vi "Sample.vi"(8 "错误输入（无错误）":errorcluster, 10 "Time and Data In":T3, 11 "Sample Settings":T1={"设备信息"={"初始索引子集"=[], "模拟信号采集通道"="Dev1", "数字-供电"="", "数字-光控"="", "光控设备"="", "光电设备分离？"=FALSE, "光谱保存路径"=path "", "环数"=0}, "测量控制"={"测头拿起"=FALSE, "起始保存"=FALSE, "测头供电"=TRUE, "测头出光"=TRUE}, "测量"={"每波长测量次数"=5, "波长"=[0, 0, 0, 0, 0, 0], "起始周期"=0, "起始测量周期"=0}, "等待"={"等待时间(s)"=0.0, "等待方式"=FALSE, "每x周期/点等待"=8, "等待时"=enum."无电无光"}, "校准"={"暗电流校准值初值"=[], "温度校准值"=[0.0, 0.0, 0.0, 0.0, 0.0, 0.0, 0.00013, 0.00013, 0.00013, 0.00013, 0.00013, 0.00013], "校准模式"=enum."逐周期"}, "图表相关"={"文件-时间"=""}, "CSM"={"CSM Name"=""}}) -> (0 "error out":errorcluster, 2 "Time and Data Out":T3)   [LabVIEW 2026, in "UI-无创.lvlib" / "Acquisition.lvlib"]
uses:
  Acquisition.lvlib
  Supports/Time and Data_OP.ctl
  Supports/Sample Settings.ctl
  <vilib>/DAQmx/read.llb/DAQmx Read (Analog 2D DBL NChan NSamp).vi
  <vilib>/Analysis/baseanly.llb/Mean (DBL).vi
  <vilib>/DAQmx/create/channels.llb/DAQmx Create Channel (AI-Voltage-Basic).vi
  <vilib>/DAQmx/configure/timing.llb/DAQmx Timing (Sample Clock).vi
  <vilib>/DAQmx/miscellaneous.llb/DAQmx Fill In Error Info.vi
  <vilib>/Analysis/NI_AALBase.lvlib
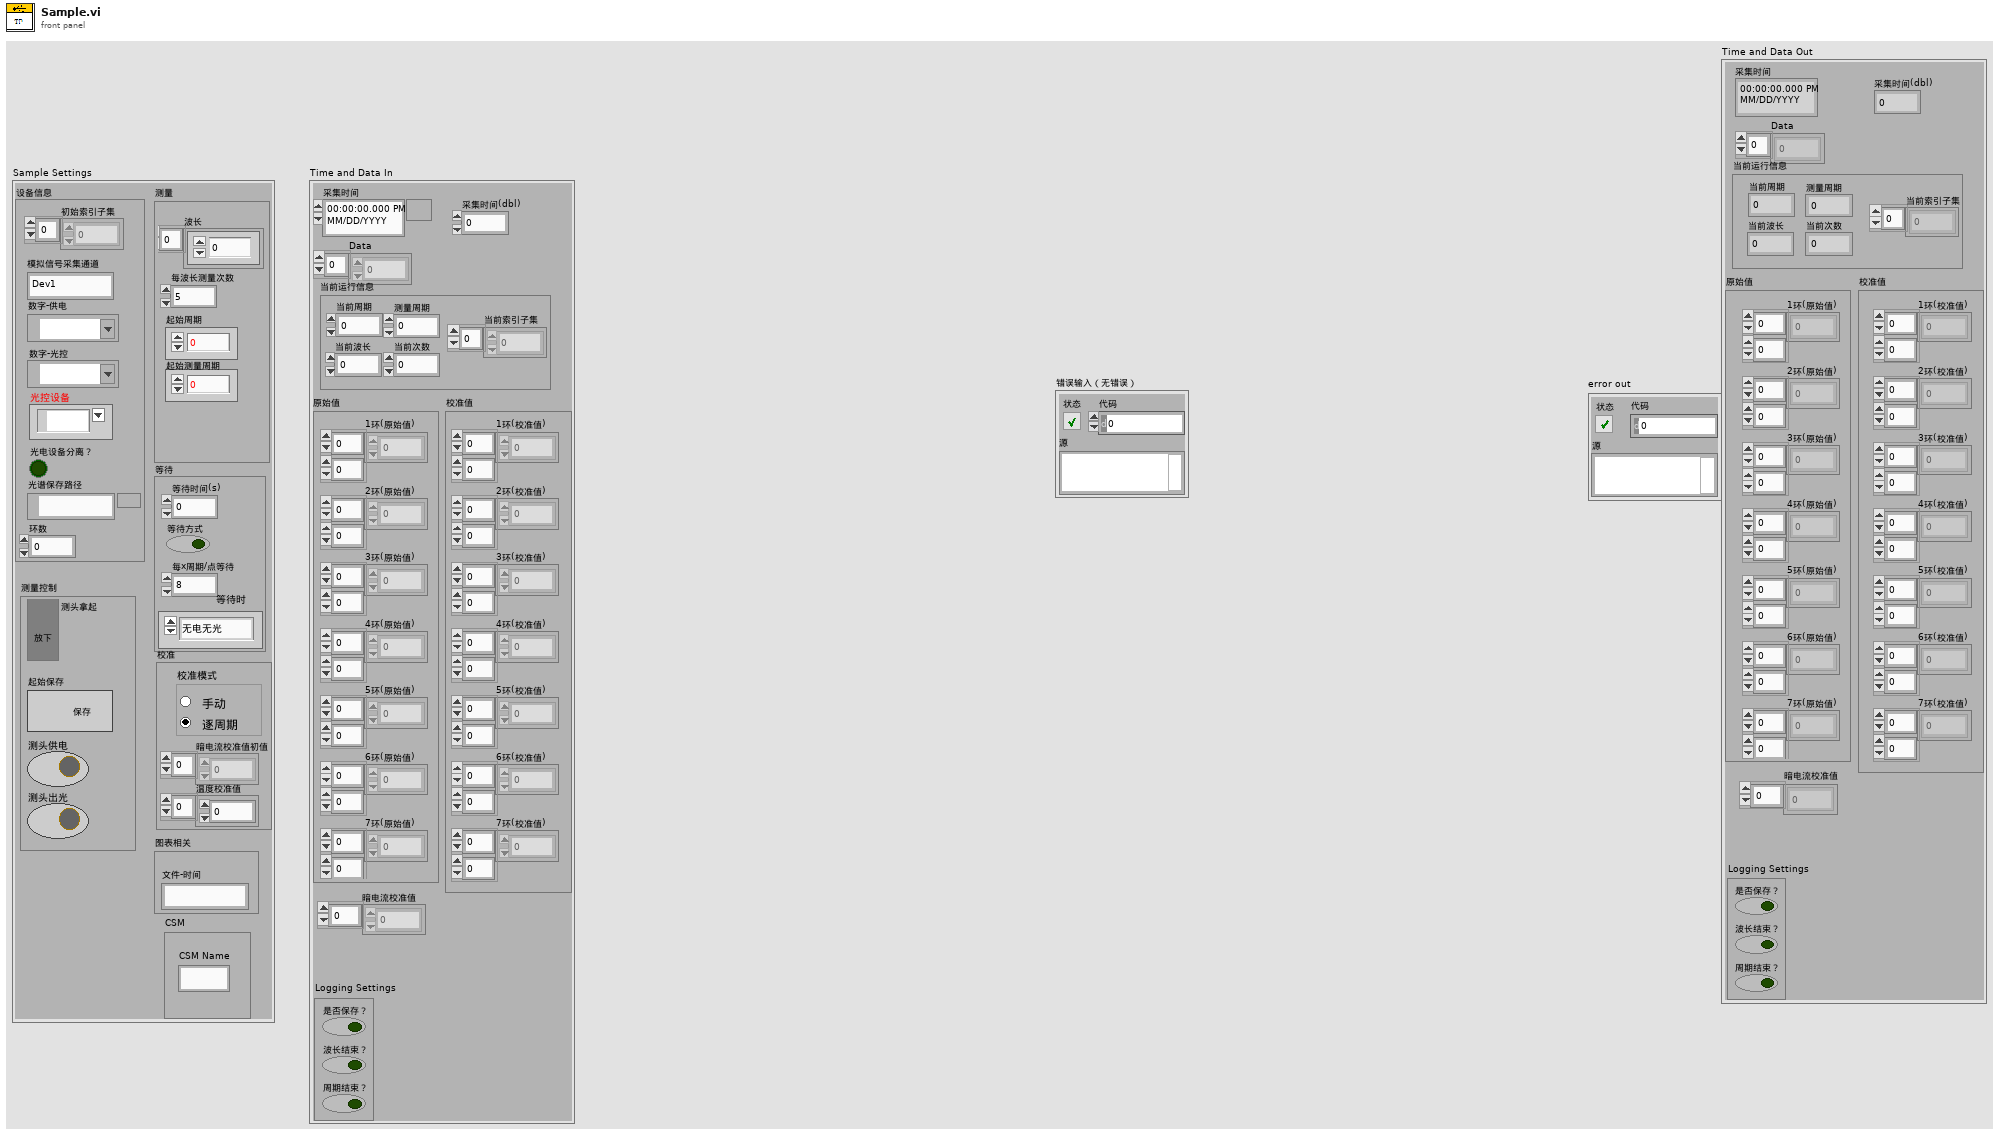
[diagram p1: front panel]
types:
  T1 = typedef "UI-无创.lvlib/Sample Settings.ctl" = cluster{"设备信息":cluster{"初始索引子集":i8[], "模拟信号采集通道":string, "数字-供电":refnum<k21>, "数字-光控":refnum<k21>, "光控设备":tag, "光电设备分离？":bool, "光谱保存路径":path, "环数":u8}, "测量控制":cluster{"测头拿起":bool, "起始保存":bool, "测头供电":bool, "测头出光":bool}, "测量":cluster{"每波长测量次数":i32, "波长":i32[], "起始周期":i32, "起始测量周期":i32}, "等待":cluster{"等待时间(s)":dbl, "等待方式":bool, "每x周期/点等待":i32, "等待时":enum16{"无电无光", "有电无光", "无电有光", "有电有光"}}, "校准":cluster{"暗电流校准值初值":dbl[], "温度校准值":dbl[], "校准模式":T2}, "图表相关":cluster{"文件-时间":string}, "CSM":cluster{"CSM Name":string}}
  T2 = typedef "UI-无创.lvlib/暗电流校准模式.ctl" = enum32{"手动", "逐周期"}
  T3 = typedef "UI-无创.lvlib/Time and Data_OP.ctl" = cluster{"采集时间":timestamp, "采集时间(dbl)":dbl, "Data":dbl[], "当前运行信息":cluster{"当前周期":i32, "当前次数":i32, "测量周期":i32, "当前索引子集":i8[], "当前波长":i32}, "暗电流校准值":dbl[], "Logging Settings":cluster{"是否保存？":bool, "波长结束？":bool, "周期结束？":bool}, "原始值":cluster{"1环(原始值)":dbl[][], "2环(原始值)":dbl[][], "3环(原始值)":dbl[][], "4环(原始值)":dbl[][], "5环(原始值)":dbl[][], "6环(原始值)":dbl[][], "7环(原始值)":dbl[][]}, "校准值":cluster{"1环(校准值)":dbl[][], "2环(校准值)":dbl[][], "3环(校准值)":dbl[][], "4环(校准值)":dbl[][], "5环(校准值)":dbl[][], "6环(校准值)":dbl[][], "7环(校准值)":dbl[][]}}
  T4 = cluster{"Time and Data In":T3, "Sample Settings":T1}
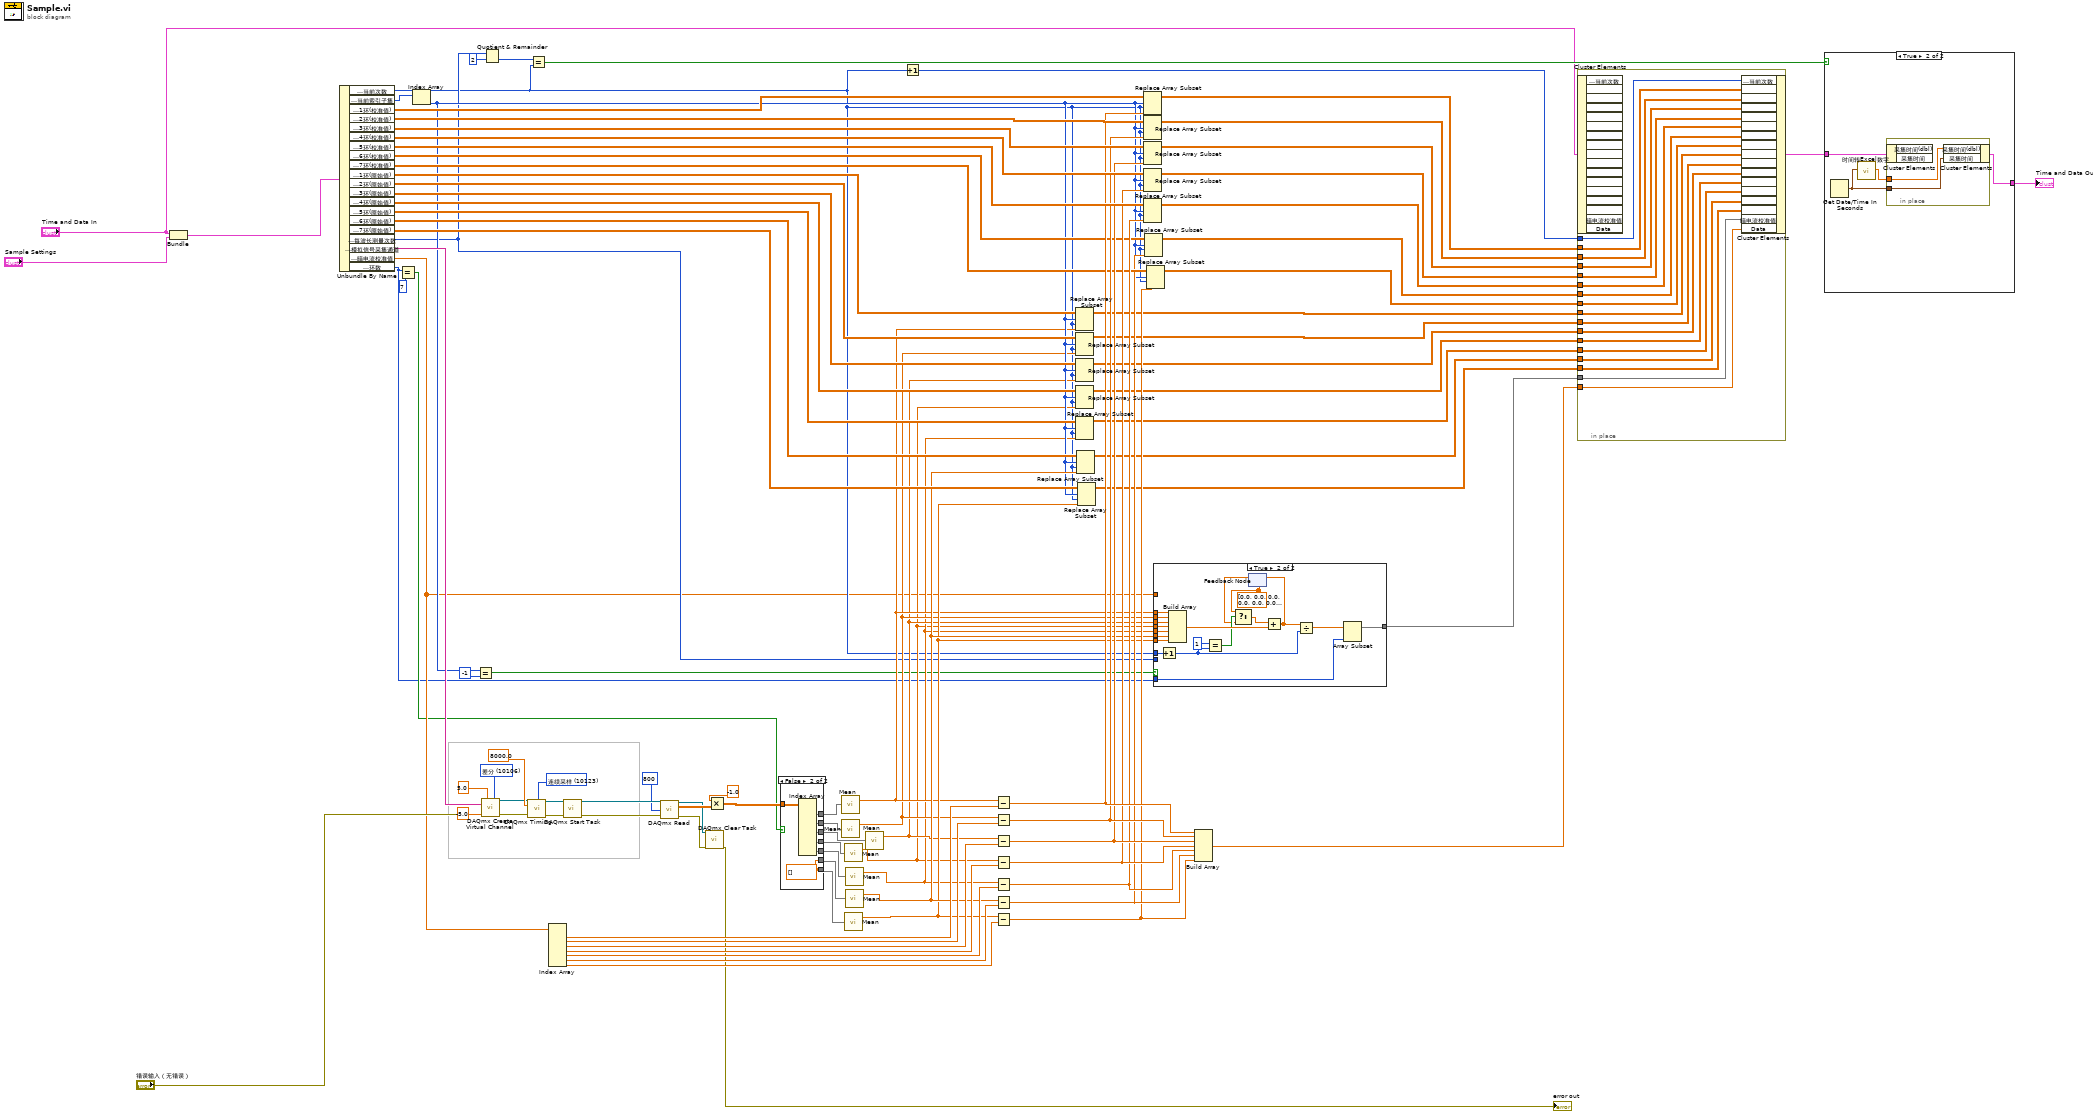
[diagram p0: block diagram]
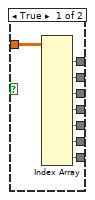
[diagram p3: hidden frame]
diagram:
  w70 = 10106 items=["默认"=-1, "RSE"=10083, "NRSE"=10078, "差分"=10106, "伪差分"=12529] ("接线端配置")
  w80 = 10123 items=["有限采样"=10178, "连续采样"=10123, "硬件定时单点"=12522] ("sample mode")
  n1 = Bundle("Time and Data In"="Time and Data In", "Sample Settings"="Sample Settings") -> (w33:T4)  [unwired: 1 in]
  n2 = Unbundle By Name(w33) -> ("Time and Data In.当前运行信息.当前次数"=w26:i32, "Time and Data In.当前运行信息.当前索引子集"=w93:i8[], "Time and Data In.校准值.1环(校准值)"=w97:dbl[][], "Time and Data In.校准值.2环(校准值)"=w96:dbl[][], "Time and Data In.校准值.3环(校准值)"=w95:dbl[][], "Time and Data In.校准值.4环(校准值)"=w94:dbl[][], "Time and Data In.校准值.5环(校准值)"=w92:dbl[][], "Time and Data In.校准值.6环(校准值)"=w56:dbl[][], "Time and Data In.校准值.7环(校准值)"=w55:dbl[][], "Time and Data In.原始值.1环(原始值)"=w52:dbl[][], "Time and Data In.原始值.2环(原始值)"=w51:dbl[][], "Time and Data In.原始值.3环(原始值)"=w50:dbl[][], "Time and Data In.原始值.4环(原始值)"=w49:dbl[][], "Time and Data In.原始值.5环(原始值)"=w48:dbl[][], "Time and Data In.原始值.6环(原始值)"=w47:dbl[][], "Time and Data In.原始值.7环(原始值)"=w46:dbl[][], "Sample Settings.测量.每波长测量次数"=w29:i32, "Sample Settings.设备信息.模拟信号采集通道"=w66:string, "Time and Data In.暗电流校准值"=w24:dbl[], "Sample Settings.设备信息.环数"=w20:u8)
  n3 = Equal?(x=w20, y=u8 7) -> (x = y?=w21:bool)
  n4 = Index Array(array=w93) -> (element=w42:i8)  [unwired: 1 in]
  n5 = Equal?(x=w42, y=-1) -> (x = y?=w35:bool)
  n6 = call-poly <vilib>:"DAQmx Create Virtual Channel.vi"("maximum value"=5.0 ("最大电压"), "minimum value"=-5.0 ("最小电压"), "input terminal configuration"=w70, "physical channels"=w66, "error in"="错误输入（无错误）") -> ("task out"=w81:refnum<k21>, "error out"=w67:errorcluster)  [unwired: 9 in]
  n7 = Quotient & Remainder(x=w29, y=2) -> (floor(x/y)=w27:i32)  [unwired: 1 out]
  n8 = call-poly <vilib>:"DAQmx Timing.vi"("task/channels in"=w81, "sample mode"=w80, "rate"=8000.0 ("采样率"), "error in"=w67) -> ("task out"=w83:refnum<k21>, "error out"=w84:errorcluster)  [unwired: 10 in]
  n9 = Equal?(x=w27, y=w26) -> (x = y?=w25:bool)
  n10 = Index Array(array=w24) -> (element #1=w89:dbl, element #2=w88:dbl, element #3=w87:dbl, element #4=w86:dbl, element #5=w85:dbl, element #6=w58:dbl, element #7=w57:dbl)  [unwired: 7 in]
  n11 = call <vilib>:"DAQmx Start Task.vi"("task/channels in"=w83, "error in"=w84) -> ("task out"=w79:refnum<k21>, "error out"=w78:errorcluster)  [unwired: 12 in]
  n12 = call-poly <vilib>:"DAQmx Read.vi"("task/channels in"=w79, "number of samples per channel"=800, "error in"=w78) -> ("task out"=w77:refnum<k21>, "data"=w91:dbl[][], "error out"=w76:errorcluster)  [unwired: 10 in]
  n13 = call <vilib>:"DAQmx Clear Task.vi"("task in"=w77, "error in"=w76) -> ("error out"=→"error out":errorcluster)  [unwired: 13 in]
  n14 = Multiply(x=-1.0, y=w91) -> (x*y=w41:dbl[][])
  n15 = case shown="False" w21 {
    tunnel: [w105 w112] -> w75
    tunnel: [w104 w111] -> w74
    tunnel: [w103 w110] -> w73
    tunnel: [w102 w109] -> w72
    tunnel: [w101 w108] -> w71
    tunnel: w41 -> [w100 w107]
    tunnel: [w99 w106] -> w60
    tunnel: [w98 w106] -> w59
    frame True {
      n16 = Index Array(array=w100) -> (element #1=w105:dbl[], element #2=w104:dbl[], element #3=w103:dbl[], element #4=w102:dbl[], element #5=w101:dbl[], element #6=w99:dbl[], element #7=w98:dbl[])  [unwired: 14 in]
    }
    frame False {
      w106 = dbl[] []
      n17 = Index Array(array=w107) -> (element #1=w112:dbl[], element #2=w111:dbl[], element #3=w110:dbl[], element #4=w109:dbl[], element #5=w108:dbl[])  [unwired: 10 in]
    }
  }
  n18 = call-poly <vilib>:"Mean.vi"("X"=w75) -> ("mean"=w40:dbl)  [unwired: 1 out]
  n19 = call-poly <vilib>:"Mean.vi"("X"=w74) -> ("mean"=w39:dbl)  [unwired: 1 out]
  n20 = call-poly <vilib>:"Mean.vi"("X"=w72) -> ("mean"=w36:dbl)  [unwired: 1 out]
  n21 = call-poly <vilib>:"Mean.vi"("X"=w59) -> ("mean"=w44:dbl)  [unwired: 1 out]
  n22 = call-poly <vilib>:"Mean.vi"("X"=w71) -> ("mean"=w37:dbl)  [unwired: 1 out]
  n23 = call-poly <vilib>:"Mean.vi"("X"=w60) -> ("mean"=w45:dbl)  [unwired: 1 out]
  n24 = call-poly <vilib>:"Mean.vi"("X"=w73) -> ("mean"=w38:dbl)  [unwired: 1 out]
  n25 = Increment(x=w26) -> (x+1=w17:i32)
  n26 = Subtract(x=w40, y=w89) -> (x-y=w65:dbl)
  n27 = Subtract(x=w39, y=w88) -> (x-y=w64:dbl)
  n28 = Subtract(x=w38, y=w87) -> (x-y=w63:dbl)
  n29 = Subtract(x=w36, y=w86) -> (x-y=w62:dbl)
  n30 = Subtract(x=w37, y=w85) -> (x-y=w61:dbl)
  n31 = Subtract(x=w45, y=w58) -> (x-y=w54:dbl)
  n32 = Subtract(x=w44, y=w57) -> (x-y=w53:dbl)
  n33 = Replace Array Subset(array=w52, new element=w40, index (row)=w42, index (col)=w26) -> (w9:dbl[][])
  n34 = Replace Array Subset(array=w51, new element=w39, index (row)=w42, index (col)=w26) -> (w8:dbl[][])
  n35 = Replace Array Subset(array=w50, new element=w38, index (row)=w42, index (col)=w26) -> (w7:dbl[][])
  n36 = Replace Array Subset(array=w49, new element=w36, index (row)=w42, index (col)=w26) -> (w6:dbl[][])
  n37 = Replace Array Subset(array=w48, new element=w37, index (row)=w42, index (col)=w26) -> (w5:dbl[][])
  n38 = Replace Array Subset(array=w47, new element=w45, index (row)=w42, index (col)=w26) -> (w4:dbl[][])
  n39 = Replace Array Subset(array=w46, new element=w44, index (row)=w42, index (col)=w26) -> (w3:dbl[][])
  n40 = Replace Array Subset(array=w97, new element=w65, index (row)=w42, index (col)=w26) -> (w16:dbl[][])
  n41 = Replace Array Subset(array=w96, new element=w64, index (row)=w42, index (col)=w26) -> (w15:dbl[][])
  n42 = Replace Array Subset(array=w95, new element=w63, index (row)=w42, index (col)=w26) -> (w14:dbl[][])
  n43 = Replace Array Subset(array=w94, new element=w62, index (row)=w42, index (col)=w26) -> (w13:dbl[][])
  n44 = Replace Array Subset(array=w92, new element=w61, index (row)=w42, index (col)=w26) -> (w12:dbl[][])
  n45 = Replace Array Subset(array=w56, new element=w54, index (row)=w42, index (col)=w26) -> (w11:dbl[][])
  n46 = Replace Array Subset(array=w55, new element=w53, index (row)=w42, index (col)=w26) -> (w10:dbl[][])
  n47 = case shown="True" w35 {
    tunnel: w40 -> [_ w132]
    tunnel: w39 -> [_ w131]
    tunnel: w38 -> [_ w130]
    tunnel: w36 -> [_ w129]
    tunnel: w37 -> [_ w128]
    tunnel: w45 -> [_ w127]
    tunnel: w44 -> [_ w126]
    tunnel: [w113 w115] -> w2
    tunnel: w24 -> [w113 _]
    tunnel: w26 -> [_ w123]
    tunnel: w29 -> [_ _]
    tunnel: w20 -> [_ w114]
    frame False {
    }
    frame True {
      w120 = dbl[] [0.0, 0.0, 0.0, 0.0, 0.0, 0.0, 0.0] ("x")
      n48 = Increment(x=w123) -> (x+1=w117:i32)
      n49 = Build Array(w132, w131, w130, w129, w128, w127, w126) -> (w125:dbl[])
      n50 = Equal?(x=1 ("y"), y=w117) -> (x = y?=w121:bool)
      n51 = feedback #1(w120) -> (w119:dbl[])
      n52 = Select(t=w120, s=w121, f=w119) -> (s? t:f=w118:dbl[])
      n53 = Add(x=w118, y=w125) -> (x+y=w124:dbl[])
      n54 = feedback-in #1(w124) -> ()
      n55 = Divide(x=w124, y=w117) -> (x/y=w116:dbl[])
      n56 = Array Subset(array=w116, length=w114) -> (w115:dbl[])  [unwired: 1 in]
    }
  }
  n57 = Build Array(w65, w64, w63, w62, w61, w54, w53) -> (w1:dbl[])
  n58 = in-place {
    in-place-border: w17 -> [w149]
    in-place-border: w16 -> [w148]
    in-place-border: w15 -> [w147]
    in-place-border: w14 -> [w146]
    in-place-border: w13 -> [w145]
    in-place-border: w12 -> [w144]
    in-place-border: w11 -> [w143]
    in-place-border: w10 -> [w142]
    in-place-border: w9 -> [w141]
    in-place-border: w8 -> [w140]
    in-place-border: w7 -> [w139]
    in-place-border: w6 -> [w138]
    in-place-border: w5 -> [w137]
    in-place-border: w4 -> [w136]
    in-place-border: w3 -> [w135]
    in-place-border: w2 -> [w134]
    in-place-border: w1 -> [w133]
    n59 = in-place-cluster #2("Time and Data In") -> ()  [unwired: 17 out]
    n60 = in-place-cluster #2("当前运行信息.当前次数"=w149, "校准值.1环(校准值)"=w148, "校准值.2环(校准值)"=w147, "校准值.3环(校准值)"=w146, "校准值.4环(校准值)"=w145, "校准值.5环(校准值)"=w144, "校准值.6环(校准值)"=w143, "校准值.7环(校准值)"=w142, "原始值.1环(原始值)"=w141, "原始值.2环(原始值)"=w140, "原始值.3环(原始值)"=w139, "原始值.4环(原始值)"=w138, "原始值.5环(原始值)"=w137, "原始值.6环(原始值)"=w136, "原始值.7环(原始值)"=w135, "暗电流校准值"=w134, "Data"=w133) -> (w18:T3)
  }
  n61 = case shown="True" w25 {
    tunnel: w18 -> [w150 w154]
    tunnel: [w150 w151] -> w30
    frame False {
    }
    frame True {
      n62 = Get Date/Time In Seconds() -> (seconds since 1Jan1904=w152:timestamp)
      n63 = call "时间转Excel数字.vi"("温湿度采集时刻"=w152) -> ("数值"=w153:dbl)  [unwired: 10 in]
      n64 = in-place {
        in-place-border: w153 -> [w156]
        in-place-border: w152 -> [w155]
        n65 = in-place-cluster #3(w154) -> ()  [unwired: 2 out]
        n66 = in-place-cluster #3("采集时间(dbl)"=w156, "采集时间"=w155) -> (w151:T3)
      }
    }
  }
  "Time and Data Out" <- w30
